vi "DiffDrivePoseEst_UpdateWithTime.vi"(4 "RightDistance":dbl, 5 "LeftSpeed":dbl, 6 "LeftDistance":dbl, 7 "RightSpeed":dbl, 9 "GyroAngle":T3={"VALUE"=0.0, "COS"=1.0, "SIN"=0.0} {"SIN" format="%13.4f"; "COS" format="%13.4f"; "VALUE" format="%13.4f"}, 10 "CurrentTimeSeconds":dbl, 11 "in DiffDrivePoseEstimate":T4={"M_VisionContR"=[], "m_nominal_dT"=0.0, "m_PrevTime_Sec"=0.0, "m_GyroOffset"={"VALUE"=0.0, "COS"=1.0, "SIN"=0.0}, "m_PrevAngle"={"VALUE"=0.0, "COS"=1.0, "SIN"=0.0}, "StartLeftEnc_M"=0.0, "StartRightEnc_M"=0.0, "m_Observer"={"m_P"=[], "m_xHat"=[], "States"=0, "Outputs"=0, "m_ContR"=[], "m_ContQ"=[], "m_SigmasF"=[], "m_dT_Sec"=0.0, "MERWE_SCALED_SIGMA_PTS"={"m_Wm"=[], "States"=0, "Alpha"=0.0, "m_Wc"=[], "Kappa"=0}, "meanFuncX"=refnum, "meanFuncY"=refnum, "residualFuncX"=refnum, "residualFuncY"=refnum, "addFuncX"=refnum, "addFuncXExtra"=variant, "residualFuncYExtra"=variant, "residualFuncXExtra"=variant, "MeanFuncYExtra"=variant, "MeanFuncXExtra"=variant, "Inputs"=0}, "Pose_Buffer"={"TimeStamps"=[], "Pose"=[], "Min_TimeStamp"=0.0, "Max_TimeStamp"=0.0, "ItemCount"=0, "MaxBufferTime"=0.0}} {"Pose_Buffer"."Pose"."ROTATION"."SIN" format="%13.4f"; "Pose_Buffer"."Pose"."ROTATION"."COS" format="%13.4f"; "Pose_Buffer"."Pose"."ROTATION"."VALUE" format="%13.4f"; "Pose_Buffer"."Pose"."TRANSLATION"."Y" format="%14.3f"; "Pose_Buffer"."Pose"."TRANSLATION"."X" format="%14.3f"; "m_PrevAngle"."SIN" format="%13.4f"; "m_PrevAngle"."COS" format="%13.4f"; "m_PrevAngle"."VALUE" format="%13.4f"; "m_GyroOffset"."SIN" format="%13.4f"; "m_GyroOffset"."COS" format="%13.4f"; "m_GyroOffset"."VALUE" format="%13.4f"}) -> (0 "Error":bool, 2 "Estimated Pose":T1 {"ROTATION"."SIN" format="%13.4f"; "ROTATION"."COS" format="%13.4f"; "ROTATION"."VALUE" format="%13.4f"; "TRANSLATION"."Y" format="%14.3f"; "TRANSLATION"."X" format="%14.3f"}, 3 "Out DiffDrivePoseEstimate":T4={"M_VisionContR"=[], "m_nominal_dT"=0.0, "m_PrevTime_Sec"=0.0, "m_GyroOffset"={"VALUE"=0.0, "COS"=1.0, "SIN"=0.0}, "m_PrevAngle"={"VALUE"=0.0, "COS"=1.0, "SIN"=0.0}, "StartLeftEnc_M"=0.0, "StartRightEnc_M"=0.0, "m_Observer"={"m_P"=[], "m_xHat"=[], "States"=0, "Outputs"=0, "m_ContR"=[], "m_ContQ"=[], "m_SigmasF"=[], "m_dT_Sec"=0.0, "MERWE_SCALED_SIGMA_PTS"={"m_Wm"=[], "States"=0, "Alpha"=0.0, "m_Wc"=[], "Kappa"=0}, "meanFuncX"=refnum, "meanFuncY"=refnum, "residualFuncX"=refnum, "residualFuncY"=refnum, "addFuncX"=refnum, "addFuncXExtra"=variant, "residualFuncYExtra"=variant, "residualFuncXExtra"=variant, "MeanFuncYExtra"=variant, "MeanFuncXExtra"=variant, "Inputs"=0}, "Pose_Buffer"={"TimeStamps"=[], "Pose"=[], "Min_TimeStamp"=0.0, "Max_TimeStamp"=0.0, "ItemCount"=0, "MaxBufferTime"=0.0}} {"Pose_Buffer"."Pose"."ROTATION"."SIN" format="%13.4f"; "Pose_Buffer"."Pose"."ROTATION"."COS" format="%13.4f"; "Pose_Buffer"."Pose"."ROTATION"."VALUE" format="%13.4f"; "Pose_Buffer"."Pose"."TRANSLATION"."Y" format="%14.3f"; "Pose_Buffer"."Pose"."TRANSLATION"."X" format="%14.3f"; "m_PrevAngle"."SIN" format="%13.4f"; "m_PrevAngle"."COS" format="%13.4f"; "m_PrevAngle"."VALUE" format="%13.4f"; "m_GyroOffset"."SIN" format="%13.4f"; "m_GyroOffset"."COS" format="%13.4f"; "m_GyroOffset"."VALUE" format="%13.4f"})   [LabVIEW 2019, in "Trajectory_Library.lvlib"]
doc: "This set of functions is deprecated. Suggest using the new Diff Drive Pose Est 2 instead.\n\nUpdates the the Unscented Kalman Filter using only wheel encoder information. Note that this should be called every loop.\n\nInputs:\n - LeftSpeed -- Left wheel speed (meters/sec)\n - RightSpeed -- Right wheel speed (meters/sec)\n - inDiffDrivePoseEst -- system data cluster\n - gyroAngle -- The current gyro angle. (radians)\n - currentTime -- Time at which this method was called, in seconds.\n - distanceLeftMeters -- The total distance travelled by the left wheel in meters. This can be the encoder reading.\n - distanceRightMeters -- The total distance travelled by the right wheel in meters. This can be the encoder reading.\n\nOutputs:\n - outDiffDrivePoseEst -- system data cluster\n - EstimatedPose -- The estimated pose of the robot in meters."
uses:
  Trajectory_Library.lvlib
  TypeDef/DIFF_DRIVE_POSE_EST.ctl
  <vilib>/Analysis/Matrix/Datatypes/RealMatrix.ctl
  TypeDef/ROTATION2D.ctl
  TypeDef/UNSCENTED_KALMAN_FILTER.ctl
  TypeDef/MERWE_SCALED_SIGMA_PTS.ctl
  TypeDef/CALLBACK_FUNC_TYPE.ctl
  TypeDef/TIME_INTERPOLATABLE_POSE2D.ctl
  TypeDef/POSE2D.ctl
  TypeDef/TRANSLATION2D.ctl
  Rotation2d_RotateBy.vi
  MatBuilder_Create.vi
  Rotation2d_UnaryMinus.vi
  VI/TimeInterpPose2d_CleanUp.vi
  Rotation2d_CreateXY.vi
  Rotation2d_CreateAngle.vi
  Util_CalcDist.vi
  <vilib>/gmath/interp.llb/Search Ordered Table.vi
  <vilib>/Analysis/Matrix/NI_Matrix.lvlib
panel:
  # "<3, 3>"
  # "State Estimate <Statess,1>"
  # "<States, States>"
  # "<States, ?>"
  # "<Statess,  States>"
  # "<Outputs, Outputs>"
  # "<?, 1>"
  # "<?, 1>"
  # "<3, 3>"
  # "State Estimate <Statess,1>"
  # "<States, States>"
  # "<States, ?>"
  # "<Statess,  States>"
  # "<Outputs, Outputs>"
  # "<?, 1>"
  # "<?, 1>"
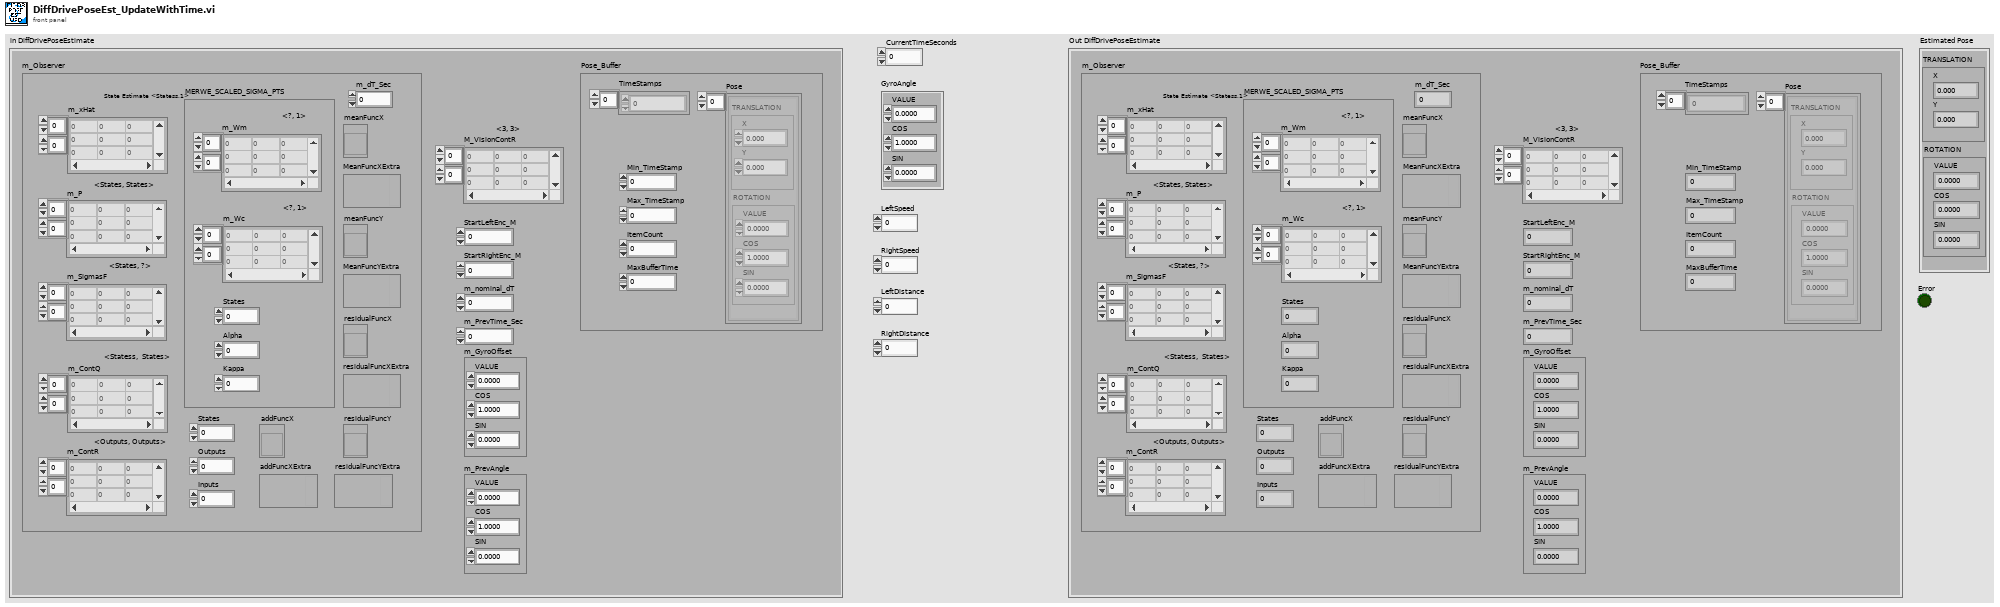
[diagram p1: front panel]
types:
  T1 = typedef "Trajectory_Library.lvlib/POSE2D.ctl" = cluster{"TRANSLATION":T2, "ROTATION":T3}
  T2 = typedef "Trajectory_Library.lvlib/TRANSLATION2D.ctl" = cluster{"X":dbl, "Y":dbl}
  T3 = typedef "Trajectory_Library.lvlib/ROTATION2D.ctl" = cluster{"VALUE":dbl, "COS":dbl, "SIN":dbl}
  T4 = typedef "Trajectory_Library.lvlib/DIFF_DRIVE_POSE_EST.ctl" = cluster{"M_VisionContR":T5, "m_nominal_dT":dbl, "m_PrevTime_Sec":dbl, "m_GyroOffset":T3, "m_PrevAngle":T3, "StartLeftEnc_M":dbl, "StartRightEnc_M":dbl, "m_Observer":T6, "Pose_Buffer":T9}
  T5 = typedef "NI_Matrix.lvlib/RealMatrix.ctl" = dbl[][]
  T6 = typedef "Trajectory_Library.lvlib/UNSCENTED_KALMAN_FILTER.ctl" = cluster{"m_P":T5, "m_xHat":T5, "States":i32, "Outputs":i32, "m_ContR":T5, "m_ContQ":T5, "m_SigmasF":T5, "m_dT_Sec":dbl, "MERWE_SCALED_SIGMA_PTS":T7, "meanFuncX":T8, "meanFuncY":T8, "residualFuncX":T8, "residualFuncY":T8, "addFuncX":T8, "addFuncXExtra":variant, "residualFuncYExtra":variant, "residualFuncXExtra":variant, "MeanFuncYExtra":variant, "MeanFuncXExtra":variant, "Inputs":i32}
  T7 = typedef "Trajectory_Library.lvlib/MERWE_SCALED_SIGMA_PTS.ctl" = cluster{"m_Wm":T5, "States":i32, "Alpha":dbl, "m_Wc":T5, "Kappa":i32}
  T8 = typedef "Trajectory_Library.lvlib/CALLBACK_FUNC_TYPE.ctl" = refnum<vi>
  T9 = typedef "Trajectory_Library.lvlib/TIME_INTERPOLATABLE_POSE2D.ctl" = cluster{"TimeStamps":dbl[], "Pose":T1[], "Min_TimeStamp":dbl, "Max_TimeStamp":dbl, "ItemCount":i32, "MaxBufferTime":dbl}
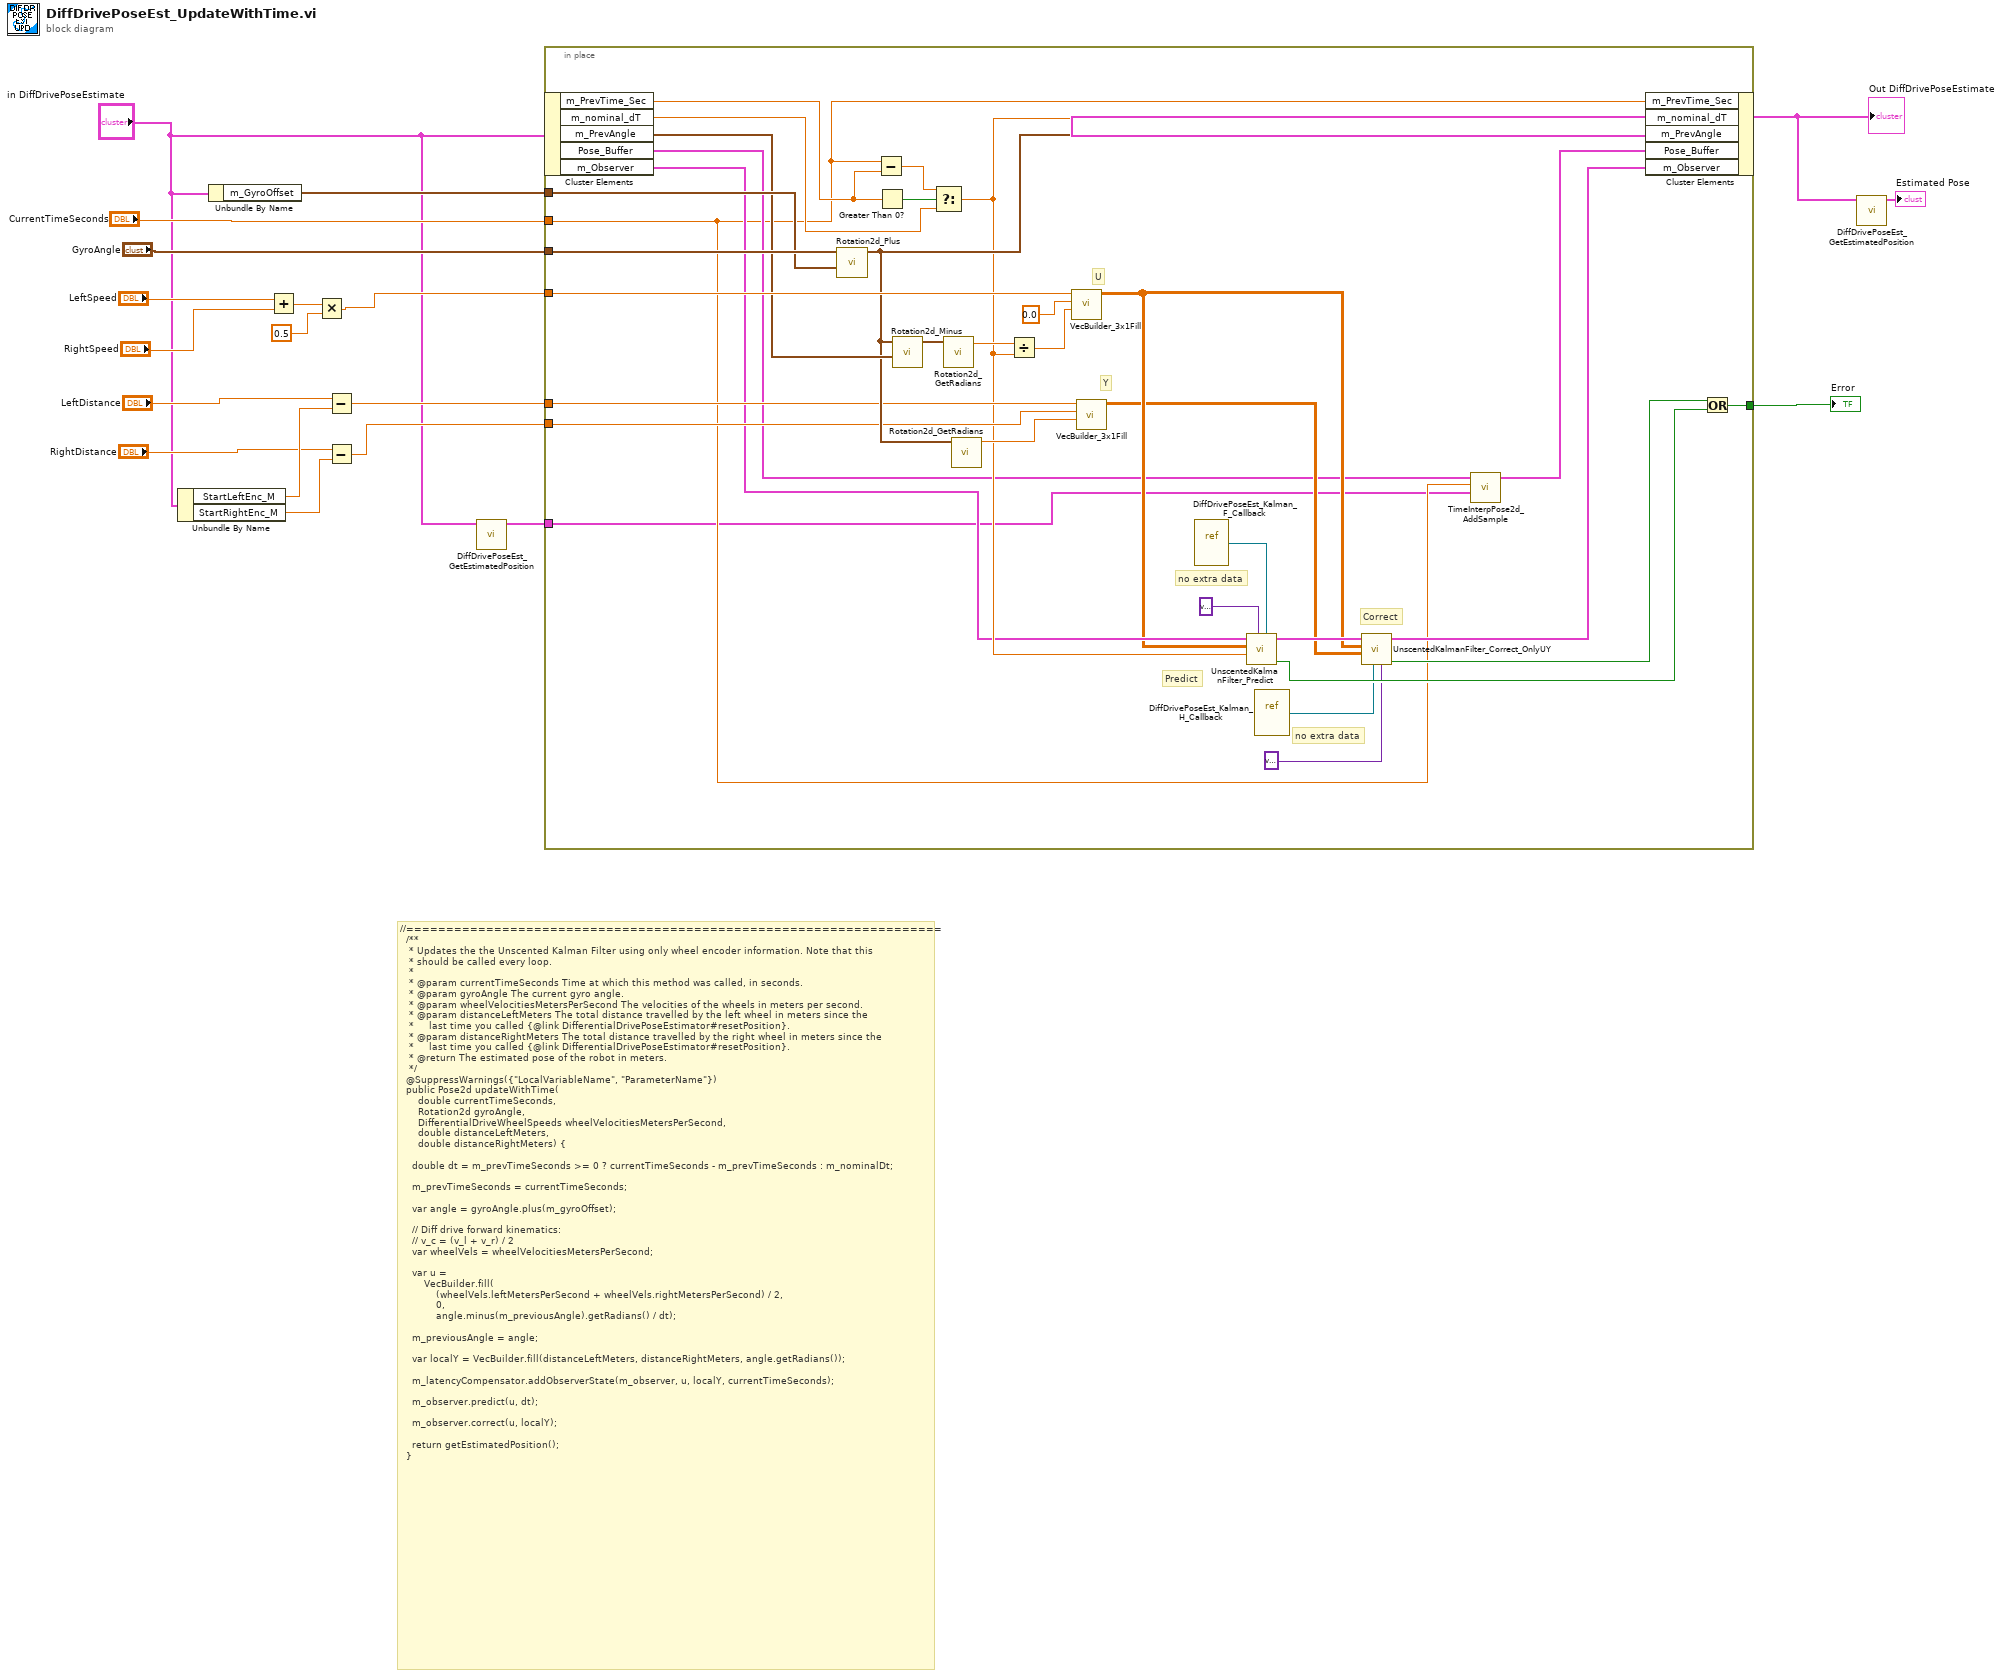
[diagram p0: block diagram]
diagram:
  # "//===================================================================\n  /**\n   * Updates the the Unscented Kalman Filter using only wheel encoder information. Note that this\n   * should be called every loop.\n   *\n   * @param currentTimeSeconds Time at which this method was called, in seconds.\n   * @param gyroAngle The current gyro angle.\n   * @param wheelVelocitiesMetersPerSecond The velocities of the wheels in meters per second.\n   * @param distanceLeftMeters The total distance travelled by the left wheel in meters since the\n   *     last time you called {@link DifferentialDrivePoseEstimator#resetPosition}.\n   * @param distanceRightMeters The total distance travelled by the right wheel in meters since the\n   *     last time you called {@link DifferentialDrivePoseEstimator#resetPosition}.\n   * @return The estimated pose of the robot in meters.\n   */\n  @SuppressWarnings({\"LocalVariableName\", \"ParameterName\"})\n  public Pose2d updateWithTime(\n      double currentTimeSeconds,\n      Rotation2d gyroAngle,\n      DifferentialDriveWheelSpeeds wheelVelocitiesMetersPerSecond,\n      double distanceLeftMeters,\n      double distanceRightMeters) {\n\n    double dt = m_prevTimeSeconds >= 0 ? currentTimeSeconds - m_prevTimeSeconds : m_nominalDt;\n\n    m_prevTimeSeconds = currentTimeSeconds;\n\n    var angle = gyroAngle.plus(m_gyroOffset);\n\n    // Diff drive forward kinematics:\n    // v_c = (v_l + v_r) / 2\n    var wheelVels = wheelVelocitiesMetersPerSecond;\n\n    var u =\n        VecBuilder.fill(\n            (wheelVels.leftMetersPerSecond + wheelVels.rightMetersPerSecond) / 2,\n            0,\n            angle.minus(m_previousAngle).getRadians() / dt);\n\n    m_previousAngle = angle;\n\n    var localY = VecBuilder.fill(distanceLeftMeters, distanceRightMeters, angle.getRadians());\n\n    m_latencyCompensator.addObserverState(m_observer, u, localY, currentTimeSeconds);\n\n    m_observer.predict(u, dt);\n\n    m_observer.correct(u, localY);\n\n    return getEstimatedPosition();\n  }"
  n1 = Unbundle By Name("in DiffDrivePoseEstimate") -> ("StartLeftEnc_M"=w6:dbl, "StartRightEnc_M"=w5:dbl)
  n2 = Unbundle By Name("in DiffDrivePoseEstimate") -> ("m_GyroOffset"=w12:T3)
  n3 = Add(x="LeftSpeed", y="RightSpeed") -> (x+y=w15:dbl)
  n4 = Multiply(x=w15, y=0.5) -> (x*y=w13:dbl)
  n5 = Subtract(x="LeftDistance", y=w6) -> (x-y=w8:dbl)
  n6 = Subtract(x="RightDistance", y=w5) -> (x-y=w7:dbl)
  n7 = call "DiffDrivePoseEst_GetEstimatedPosition.vi"("in DiffDrivePoseEstimate"="in DiffDrivePoseEstimate") -> ("Estimated Pose"=w1:T1)  [unwired: 10 in]
  n8 = in-place {
    in-place-border: "CurrentTimeSeconds" -> [w21]
    in-place-border: "GyroAngle" -> [w49]
    in-place-border: w13 -> [w48]
    in-place-border: w12 -> [w46]
    in-place-border: w8 -> [w39]
    in-place-border: w7 -> [w38]
    in-place-border: [w33] -> w9
    in-place-border: w1 -> [w20]
    # "Correct"
    # "Predict"
    # "no extra data"
    # "no extra data"
    # "Y"
    # "U"
    n9 = in-place-cluster #1("in DiffDrivePoseEstimate") -> ("m_PrevTime_Sec"=w51:dbl, "m_nominal_dT"=w43:dbl, "m_PrevAngle"=w45:T3, "Pose_Buffer"=w23:T9, "m_Observer"=w26:T6)
    n10 = call "Rotation2d_Plus.vi"("other ROTATION"=w46, "in ROTATION"=w49) -> ("out ROTATION"=w40:T3)  [unwired: 9 in]
    n11 = Subtract(x=w21, y=w51) -> (x-y=w50:dbl)
    n12 = Greater Than 0?(x=w51) -> (x > 0?=w52:bool)
    n13 = call "Rotation2d_Minus.vi"("other ROTATION"=w45, "in ROTATION"=w40) -> ("out ROTATION"=w44:T3)  [unwired: 9 in]
    n14 = Select(t=w50, s=w52, f=w43) -> (s? t:f=w32:dbl)
    n15 = call "Rotation2d_GetRadians.vi"("in ROTATION"=w44) -> ("AngleRadians"=w42:dbl)  [unwired: 10 in]
    n16 = call "Rotation2d_GetRadians.vi"("in ROTATION"=w40) -> ("AngleRadians"=w37:dbl)  [unwired: 10 in]
    n17 = Divide(x=w42, y=w32) -> (x/y=w41:dbl)
    n18 = call "VecBuilder_3x1Fill.vi"("R2"=w41, "R1"=0.0, "R0"=w48) -> ("output matrix"=w25:T5)  [unwired: 8 in]
    n19 = call "VecBuilder_3x1Fill.vi"("R2"=w37, "R1"=w38, "R0"=w39) -> ("output matrix"=w24:T5)  [unwired: 8 in]
    n20 = vi-ref "DiffDrivePoseEst_Kalman_F_Callback.vi"() -> (w31:refnum<vi>)
    n21 = call "UnscentedKalmanFilter_Predict.vi"("f_Func"=w31, "F_Func_ExtraData"=variant, "dT_Seconds"=w32, "U"=w25, "in UnscentedKalmanFiilter"=w26) -> ("Error"=w34:bool, "out UnscentedKalmanFiilter"=w36:T6)  [unwired: 5 in]
    n22 = vi-ref "DiffDrivePoseEst_Kalman_H_Callback.vi"() -> (w29:refnum<vi>)
    n23 = call "UnscentedKalmanFilter_Correct_OnlyUY.vi"("H_ExtraData"=variant ("F_Func_ExtraData"), "H_Func"=w29, "Y"=w24, "U"=w25, "in UnscentedKalmanFiilter"=w36) -> ("Error"=w35:bool, "out UnscentedKalmanFiilter"=w27:T6)  [unwired: 5 in]
    n24 = call "TimeInterpPose2d_AddSample.vi"("Pose"=w20, "TimeStamp"=w21, "in TimeInterpPose"=w23) -> ("out TimeInterpPose"=w22:T9)  [unwired: 7 in, 1 out]
    n25 = in-place-cluster #1("m_PrevTime_Sec"=w21, "m_nominal_dT"=w32, "m_PrevAngle"=w40, "Pose_Buffer"=w22, "m_Observer"=w27) -> (w11:T4)
    n26 = Or(x=w35, y=w34) -> (x .or. y?=w33:bool)
  }
  "Out DiffDrivePoseEstimate" <- w11
  "Error" <- w9
  n27 = call "DiffDrivePoseEst_GetEstimatedPosition.vi"("in DiffDrivePoseEstimate"=w11) -> ("Estimated Pose"=→"Estimated Pose":T1)  [unwired: 10 in]
